vi "set TurnTable Parameter.vi"(8 "error in (no error)":errorcluster, 10 "Turn Table Info":T1 {"Target Angle" min=0.0 max=360.0}, 11 "AUDIX EM1000 in":refnum<class "AUDIX EM1000.lvclass">) -> (0 "error out":errorcluster, 3 "AUDIX EM1000 out":refnum<class "AUDIX EM1000.lvclass">)   [LabVIEW 2023, in "Turn Table and Mast.lvlib" / "AUDIX EM1000.lvclass"]
uses:
  AUDIX EM1000.lvclass
  AUDIX EM1000.lvclass/AUDIX EM1000.ctl
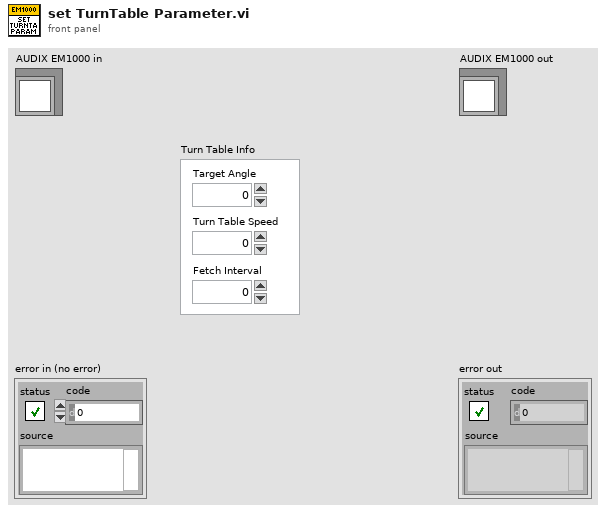
[diagram p1: front panel]
types:
  T1 = cluster{"Target Angle":dbl, "Turn Table Speed":i32, "Fetch Interval":i32}
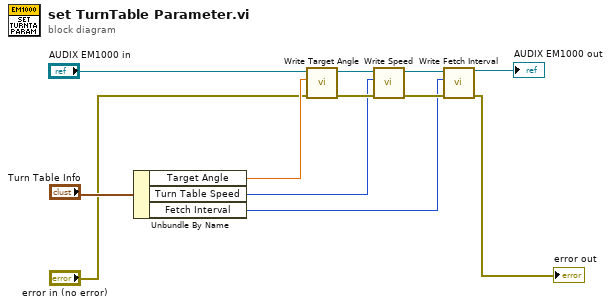
[diagram p0: block diagram]
diagram:
  n1 = Unbundle By Name("Turn Table Info") -> ("Target Angle"=w10:dbl, "Turn Table Speed"=w7:i32, "Fetch Interval"=w4:i32)
  n2 = call "Write Target Angle.vi"("error in (no error)"="error in (no error)", "Target Angle"=w10, "AUDIX EM1000 in"="AUDIX EM1000 in") -> ("error out"=w8:errorcluster, "AUDIX EM1000 out"=w9:refnum<class "AUDIX EM1000.lvclass">)  [unwired: 7 in]
  n3 = call "Write Speed.vi"("error in (no error)"=w8, "Speed"=w7, "AUDIX EM1000 in"=w9) -> ("error out"=w5:errorcluster, "AUDIX EM1000 out"=w6:refnum<class "AUDIX EM1000.lvclass">)  [unwired: 7 in]
  n4 = call "Write Fetch Interval.vi"("error in (no error)"=w5, "Fetch Interval"=w4, "AUDIX EM1000 in"=w6) -> ("error out"=→"error out":errorcluster, "AUDIX EM1000 out"=→"AUDIX EM1000 out":refnum<class "AUDIX EM1000.lvclass">)  [unwired: 7 in]
